vi "Labo03_PT100_ AprèsEtalonage.vi"() -> ()   [LabVIEW 2021]
uses:
  <instrlib>/Agilent 3446X Series/Public/Data/Read (Single Point).vi
  <vilib>/Utility/TradDaqScaling.llb/Convert RTD Reading (scaler).vi
  <instrlib>/Agilent 3446X Series/Agilent 3446X Series.lvlib
panel:
  out "Waveform Chart":sgl(graph)
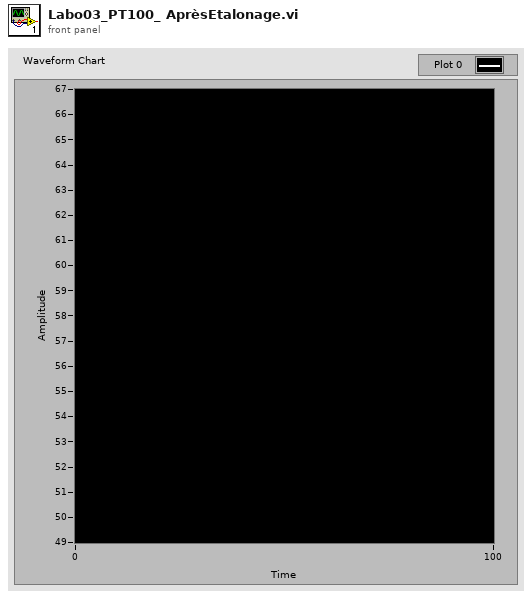
[diagram p1: front panel]
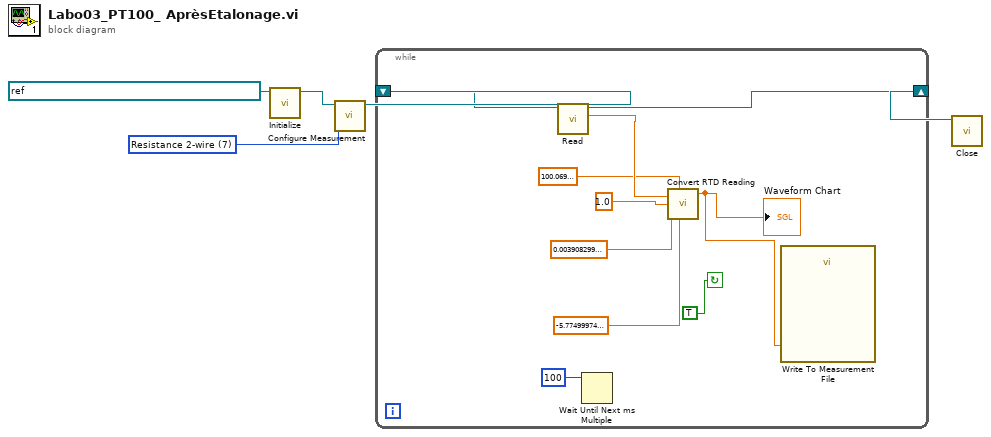
[diagram p0: block diagram]
diagram:
  w1 = 7 items=["Continuity", "Current AC", "Current DC", "Diode", "Frequency", "Resistance 4-wire", "Period", "Resistance 2-wire", "Temperature", "Voltage AC", "Voltage DC", "Voltage DC Ratio", "Capacitance"] ("Measurement Function (10: Voltage DC)")
  n1 = call <instrlib>:"Initialize.vi"("VISA resource name"=refnum<visa-resource-name> "USB0::0x2A8D::0x1601::MY53102179::INSTR") -> ("VISA resource name out"=w3:refnum<visa-resource-name>)  [unwired: 9 in, 1 out]
  n2 = call <instrlib>:"Configure Measurement.vi"("Measurement Function (10: Voltage DC)"=w1, "VISA resource name"=w3) -> ("VISA resource name out"=w4:refnum<visa-resource-name>)  [unwired: 8 in, 1 out]
  n3 = while {
    shift-right: [w15] -> w5
    shift-left: w4 -> [w14]
    stop <- TRUE continue-if-true
    n4 = call-poly <instrlib>:"Read.vi"("VISA resource name"=w14) -> ("Measurement"=w11:dbl, "VISA resource name out"=w15:refnum<visa-resource-name>)  [unwired: 8 in, 1 out]
    n5 = Wait Until Next ms Multiple(millisecond multiple=100) -> ()  [unwired: 1 out]
    n6 = call-poly <vilib>:"Convert RTD Reading.vi"("RTDvolts"=w11, "Ro"=sgl 100.07, "Iex"=sgl 1.0, "A"=sgl 0.0039083, "B"=sgl -5.775e-07) -> ("RTDtemp"=w6:sgl)  [unwired: 2 in]
    "Waveform Chart" <- w6
    n7 = call "Write To Measurement File"("Signals"=w6) -> ()  [unwired: 16 in, 3 out]
  }
  n8 = call <instrlib>:"Close.vi"("VISA resource name"=w5) -> ()  [unwired: 10 in, 1 out]
